vi "query Marker Value.vi"(8 "error in (no error)":errorcluster, 10 "Marker Index":i32=1 min=1, 11 "Keysight 9020A in":refnum<class "Keysight 9020A.lvclass">) -> (0 "error out":errorcluster, 2 "Marker Value":T1 {"X-axis" format="%#_6p"}, 3 "Keysight 9020A out":refnum<class "Keysight 9020A.lvclass">)   [LabVIEW 2023, in "Spectrum Analyzer.lvlib" / "Keysight 9020A.lvclass"]
uses:
  Keysight 9020A.lvclass
  TYPE DEFINITION/TYPE Marker Value.ctl
  Keysight 9020A.lvclass/Keysight 9020A.ctl
  Spectrum Analyzer.lvlib
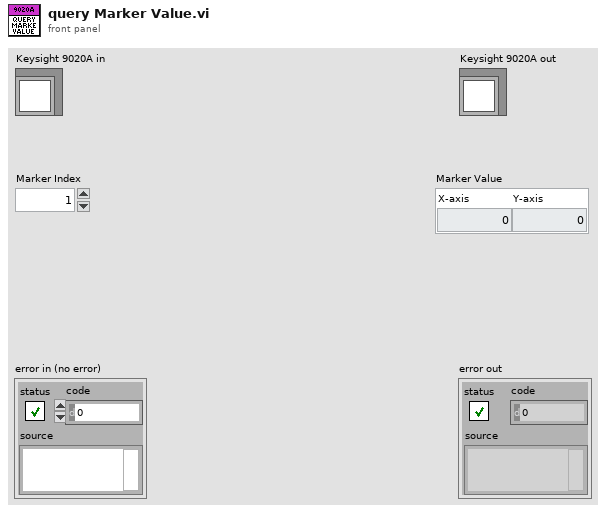
[diagram p1: front panel]
types:
  T1 = typedef "Spectrum Analyzer.lvlib/TYPE Marker Value.ctl" = cluster{"X-axis":dbl, "Y-axis":dbl}
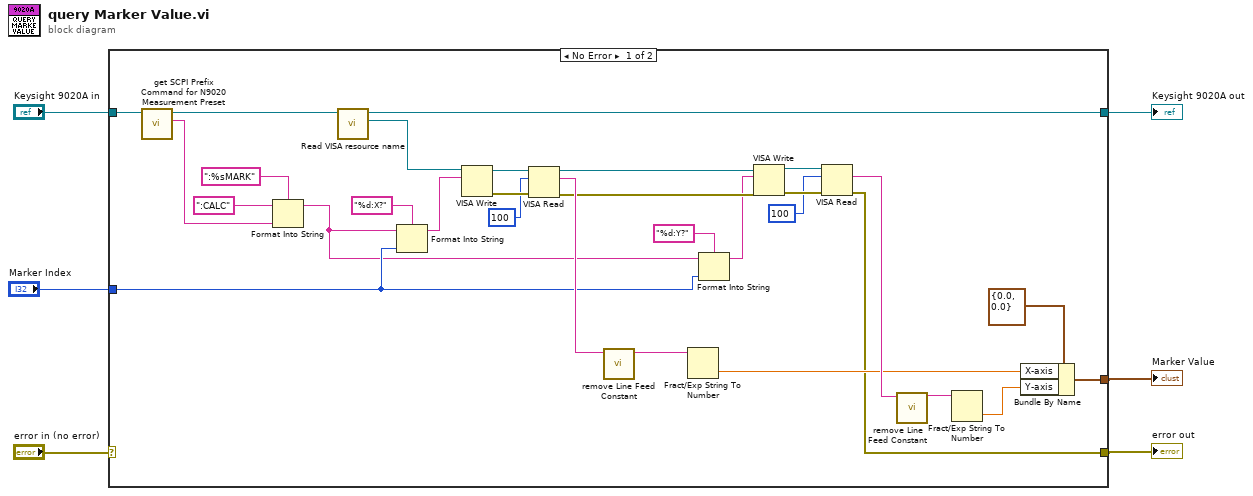
[diagram p0: block diagram]
diagram:
  n1 = case shown="No Error" "error in (no error)" {
    selector: "error in (no error)" -> [_ w37]
    tunnel: "Keysight 9020A in" -> [w9 w38]
    tunnel: [w36 w38] -> w5
    tunnel: [w20 w37] -> w3
    tunnel: [w19 _] -> w2
    tunnel: "Marker Index" -> [w13 _]
    frame No Error {
      n2 = call "get SCPI Prefix Command for N9020 Measurement Preset.vi"("Keysight 9020A in"=w9) -> ("SCPI Prefix Command"=w10:string, "Keysight 9020A out"=w8:refnum<class "Keysight 9020A.lvclass">)  [unwired: 8 in, 1 out]
      n3 = Format Into String(format string=":%sMARK", initial string=":CALC", w10) -> (resulting string=w7:string)  [unwired: 1 in, 1 out]
      n4 = call "Read VISA resource name.vi"("Keysight 9020A in"=w8) -> ("VISA resource name"=w21:refnum<visa-resource-name>, "Keysight 9020A out"=w36:refnum<class "Keysight 9020A.lvclass">)  [unwired: 8 in, 1 out]
      n5 = Format Into String(format string="%d:X?", initial string=w7, w13) -> (resulting string=w16:string)  [unwired: 1 in, 1 out]
      n6 = VISA Write(VISA resource name=w21, write buffer=w16) -> (VISA resource name out=w35:refnum<visa-resource-name>, error out=w34:errorcluster)  [unwired: 1 in, 1 out]
      n7 = VISA Read(VISA resource name=w35, byte count=u32 100, error in (no error)=w34) -> (VISA resource name out=w31:refnum<visa-resource-name>, read buffer=w32:string, error out=w30:errorcluster)  [unwired: 1 out]
      n8 = call "remove Line Feed Constant.vi"("Input String"=w32) -> ("Line Feed Removed String"=w25:string)  [unwired: 10 in]
      n9 = Fract/Exp String To Number(string=w25) -> (number=w24:dbl)  [unwired: 3 in, 1 out]
      n10 = Format Into String(format string="%d:Y?", initial string=w7, w13) -> (resulting string=w14:string)  [unwired: 1 in, 1 out]
      n11 = VISA Write(VISA resource name=w31, write buffer=w14, error in (no error)=w30) -> (VISA resource name out=w29:refnum<visa-resource-name>, error out=w28:errorcluster)  [unwired: 1 out]
      n12 = VISA Read(VISA resource name=w29, byte count=u32 100, error in (no error)=w28) -> (read buffer=w26:string, error out=w20:errorcluster)  [unwired: 2 out]
      n13 = call "remove Line Feed Constant.vi"("Input String"=w26) -> ("Line Feed Removed String"=w23:string)  [unwired: 10 in]
      n14 = Fract/Exp String To Number(string=w23) -> (number=w22:dbl)  [unwired: 3 in, 1 out]
      n15 = Bundle By Name(cluster=T1 {"X-axis"=0.0, "Y-axis"=0.0} ("Marker Value 2"), "X-axis"=w24, "Y-axis"=w22) -> (w19:T1)
    }
    frame Error {
    }
  }
  "error out" <- w3
  "Keysight 9020A out" <- w5
  "Marker Value" <- w2
